vi "Set Tool Annotations.vi"(8 "error in":errorcluster, 10 "annotations":T1, 11 "tool entry":string) -> (0 "error out":errorcluster, 3 "tool entry out":string)   [LabVIEW 2020, in "MCP Server.lvlib"]
doc: "Adds the behaviour hints of a tool to its tools/list entry, for Complete Tool Entry.vi. Every hint that is set (true or false) goes into annotations under its MCP name (readOnlyHint, destructiveHint, idempotentHint, openWorldHint). Hints that are not set are left out, so the client applies the MCP default. When no hint is set the entry gets no annotations."
uses:
  MCP Server.lvlib
  <vilib>/JDP Science/JSONtext/support/Format JSON Object.vi
  <vilib>/JDP Science/JSONtext/JSONtext.lvlib
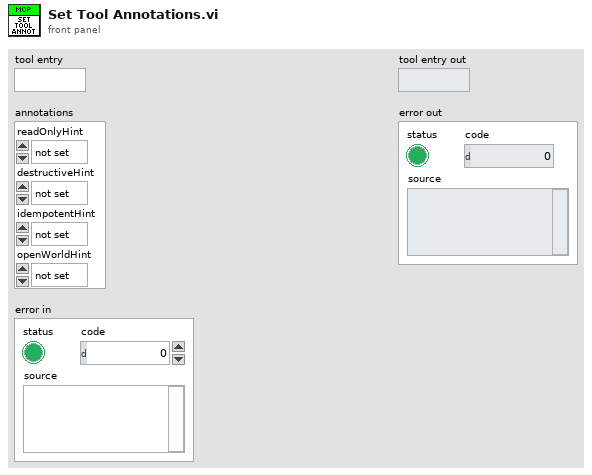
[diagram p1: front panel]
types:
  T1 = cluster{"readOnlyHint":enum16{"not set", "true", "false"}, "destructiveHint":enum16{"not set", "true", "false"}, "idempotentHint":enum16{"not set", "true", "false"}, "openWorldHint":enum16{"not set", "true", "false"}}
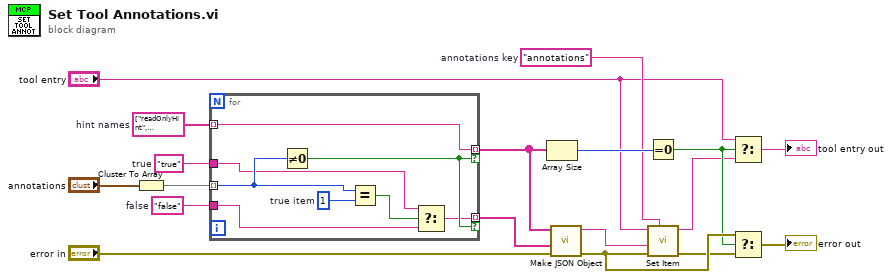
[diagram p0: block diagram]
diagram:
  w14 = "false"  # false
  w15 = "true"  # true
  w16 = string[] ["readOnlyHint", "destructiveHint", "idempotentHint", "openWorldHint"]  # hint names
  w8 = "annotations"  # annotations key
  n1 = Cluster To Array(cluster="annotations") -> (array=w17:enum16{"not set", "true", "false"}[])
  n2 = for {
    tunnel: w17 -> [w26] mode=indexing
    tunnel: w16 -> [w21] mode=indexing
    tunnel: w15 -> [w24]
    tunnel: w14 -> [w22]
    tunnel: [w21] -> w12 mode=indexing if=w20
    tunnel: [w19] -> w11 mode=indexing if=w20
    w25 = u16 1  # true item
    n3 = Not Equal To 0?(x=w26) -> (x != 0?=w20:bool)
    n4 = Equal?(x=w26, y=w25) -> (x = y?=w23:bool)
    n5 = Select(t=w24, s=w23, f=w22) -> (s? t:f=w19:string)
  }
  n6 = Array Size(array=w12) -> (size(s)=w13:i32)
  n7 = call <vilib>:"Make JSON Object.vi"("error in (no error)"="error in", "JSON Items"=w11, "Item Names"=w12) -> ("error out"=w7:errorcluster, "<JSON>"=w9:string)  [unwired: 7 in]
  n8 = Equal To 0?(x=w13) -> (x = 0?=w4:bool)
  n9 = call <vilib>:"Set Item.vi"("$Path or Item Name"=w8, "error in (no error)"=w7, "JSON to Insert"=w9, "JSON"="tool entry") -> ("error out"=w6:errorcluster, "<JSON>"=w3:string)  [unwired: 4 in, 1 out]
  n10 = Select(t="tool entry", s=w4, f=w3) -> (s? t:f=→"tool entry out":string)
  n11 = Select(t=w7, s=w4, f=w6) -> (s? t:f=→"error out":errorcluster)
